vi "UsesLlb.vi"(0 "x":dbl) -> (4 "y":dbl)   [LabVIEW 2026]
doc: "Test fixture: calls two VIs in an LLB."
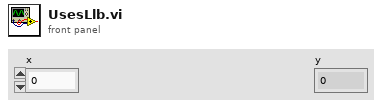
[diagram p1: front panel]
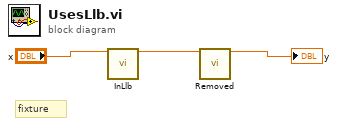
[diagram p0: block diagram]
diagram:
  # "fixture"
  n1 = call "InLlb.vi"("x"="x") -> ("y"=w2:dbl)  [unwired: 14 in]
  n2 = call "Removed.vi"("x"=w2) -> ("y"=→"y":dbl)  [unwired: 14 in]
